vi "StringInputKeyboardSimulation_Tests.vi"(11 "error in":errorcluster) -> (15 "error out":errorcluster)   [LabVIEW 2016, in "DronaTest.lvlib"]
uses:
  DronaTest.lvlib
  APIs/Stimulus/KeyBoardSimulation/KeyboardSimulationForStringInput.vi
  APIs/Assert/AssertControlValue/Equal.vi
  <vilib>/addons/_JKI Toolkits/Caraya/classes/Test/Test.lvclass
  Drona.lvlib
  APIs/Assert/AssertControlValue/AssertControlValue.lvlib
  APIs/Stimulus/KeyBoardSimulation/KeyboardSimulation.lvlib
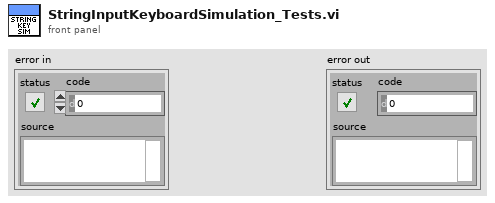
[diagram p1: front panel]
types:
  T1 = enum16{"Type all possible letters in keyboard", "TypeNegative25_ControlValueShouldBeNegative25", "Type255_ControlValueCoerceTo100", "TypeNegative257_ControlValueCoerceToNegative100"}[]
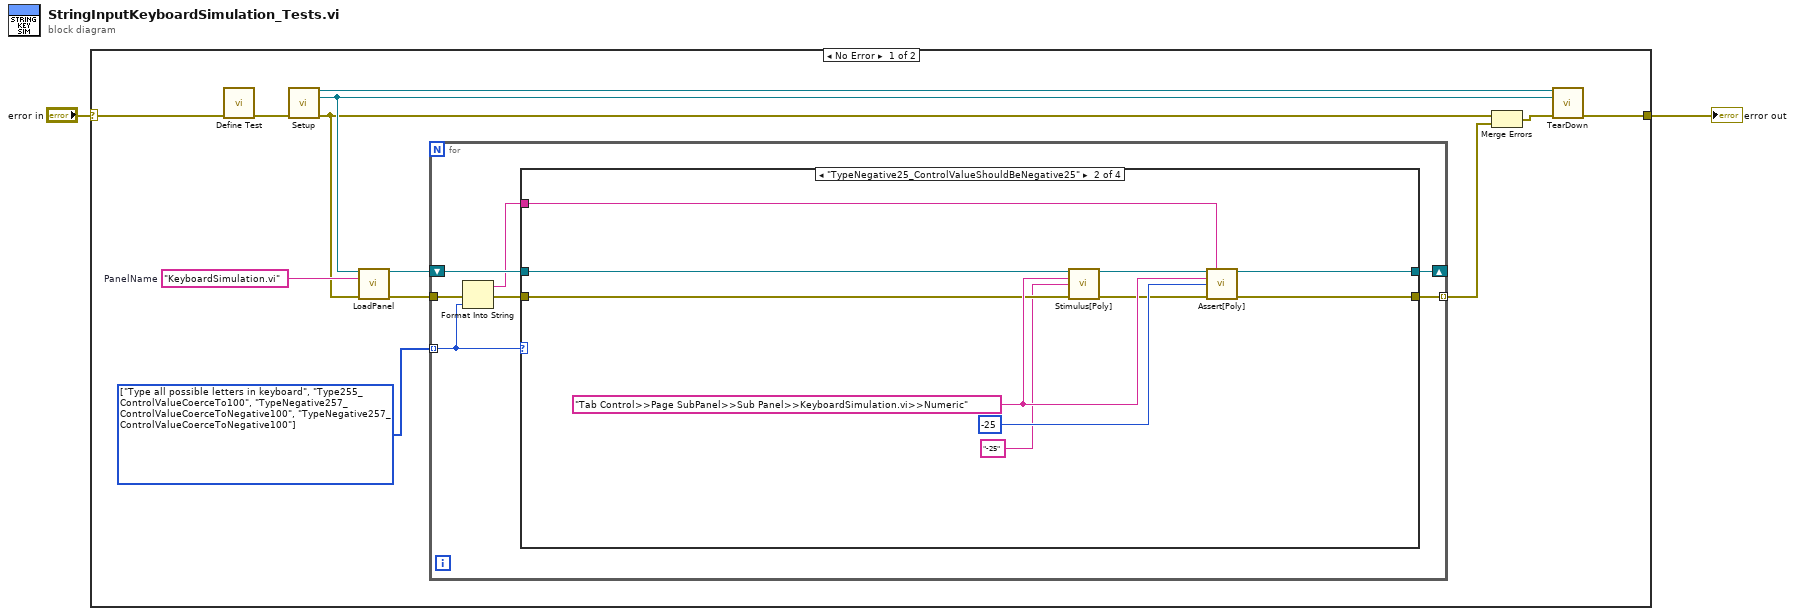
[diagram p0: block diagram]
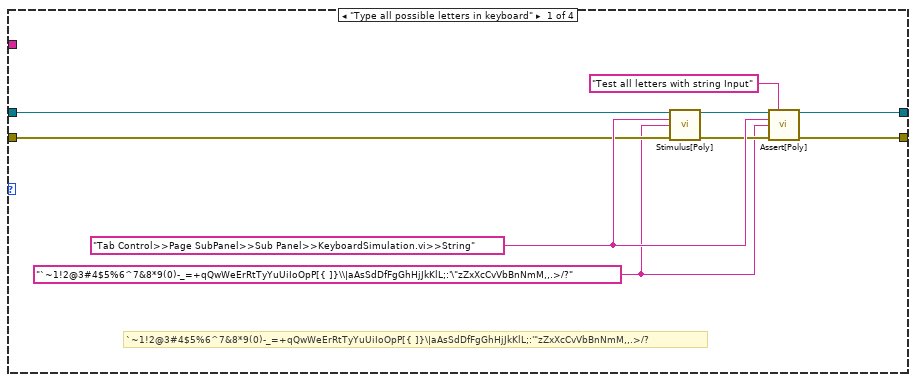
[diagram p2: hidden frame]
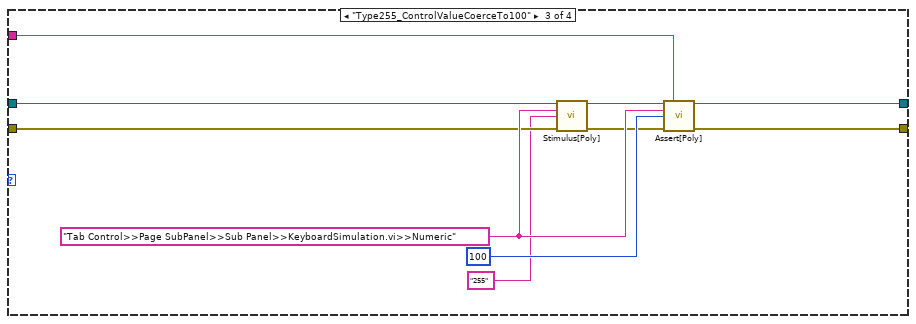
[diagram p3: hidden frame]
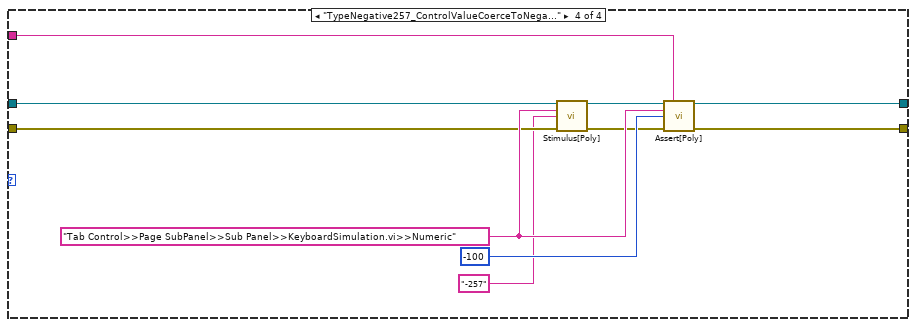
[diagram p4: hidden frame]
diagram:
  n1 = case shown="No Error" "error in" {
    selector: "error in" -> [w14 w61]
    tunnel: [w6 w61] -> w1
    frame No Error {
      w12 = T1 [enum."Type all possible letters in keyboard", enum."Type255_ControlValueCoerceTo100", enum."TypeNegative257_ControlValueCoerceToNegative100", enum."TypeNegative257_ControlValueCoerceToNegative100"] items=["Type all possible letters in keyboard", "TypeNegative25_ControlValueShouldBeNegative25", "Type255_ControlValueCoerceTo100", "TypeNegative257_ControlValueCoerceToNegative100"] ("TestCases")
      w13 = "KeyboardSimulation.vi"  # PanelName
      n2 = call <vilib>:"Define Test.vi"("error in (no error)"=w14) -> ("error out"=w8:errorcluster)  [unwired: 9 in, 1 out]
      n3 = call "Setup.vi"("error in"=w8) -> ("Application Ref"=w5:refnum<vi>, "VI out"=w4:refnum<vi>, "error out"=w3:errorcluster)  [unwired: 12 in]
      n4 = call "LoadPanel.vi"("VI in"=w4, "Item Name"=w13, "error in"=w3) -> ("VI out"=w9:refnum<vi>, "error out"=w11:errorcluster)  [unwired: 11 in]
      n5 = for {
        tunnel: w12 -> [w16] mode=indexing
        shift-right: [w20] -> _
        shift-left: w9 -> [w21]
        tunnel: w11 -> [w19]
        tunnel: [w18] -> w10 mode=indexing
        n6 = Format Into String(error in=w19, w16) -> (resulting string=w15:string, error out=w17:errorcluster)  [unwired: 2 in]
        n7 = case shown="\"TypeNegative25_ControlValueShouldBeNegative25\"" w16 {
          tunnel: [w27 w36 w46 w56] -> w18
          tunnel: w21 -> [w26 w34 w44 w54]
          tunnel: [w25 w35 w45 w55] -> w20
          tunnel: w17 -> [w24 w33 w43 w53]
          tunnel: w15 -> [_ w32 w42 w52]
          frame "Type all possible letters in keyboard" {
            w22 = "`~1!2@3#4$5%6^7&8*9(0)-_=+qQwWeErRtTyYuUiIoOpP[{ ]}\\|aAsSdDfFgGhHjJkKlL;:'\"zZxXcCvVbBnNmM,,.>/?" ("Control Path")
            w30 = "Tab Control>>Page SubPanel>>Sub Panel>>KeyboardSimulation.vi>>String" ("Control Path")
            # "`~1!2@3#4$5%6^7&8*9(0)-_=+qQwWeErRtTyYuUiIoOpP[{ ]}\\|aAsSdDfFgGhHjJkKlL;:'\"zZxXcCvVbBnNmM,,.>/?"
            n8 = call-poly "Stimulus[Poly].vi"("VI Reference In"=w26, "Control Path"=w30, "String Value"=w22, "Error In"=w24) -> ("VI Reference Out"=w29:refnum<vi>, "Error Out"=w28:errorcluster)  [unwired: 10 in]
            n9 = call-poly "Assert[Poly].vi"("VI Reference In"=w29, "Test Label"="Test all letters with string Input", "Control Path"=w30, "Control Value"=w22, "Error In"=w28) -> ("VI Reference Out"=w25:refnum<vi>, "Error Out"=w27:errorcluster)  [unwired: 8 in, 1 out]
          }
          frame "TypeNegative25_ControlValueShouldBeNegative25" {
            w39 = "Tab Control>>Page SubPanel>>Sub Panel>>KeyboardSimulation.vi>>Numeric" ("Control Path")
            n10 = call-poly "Stimulus[Poly].vi"("VI Reference In"=w34, "Control Path"=w39, "String Value"="-25" ("string"), "Error In"=w33) -> ("VI Reference Out"=w37:refnum<vi>, "Error Out"=w38:errorcluster)  [unwired: 10 in]
            n11 = call-poly "Assert[Poly].vi"("VI Reference In"=w37, "Test Label"=w32, "Control Path"=w39, "Control Value"=-25 ("Control Path"), "Error In"=w38) -> ("VI Reference Out"=w35:refnum<vi>, "Error Out"=w36:errorcluster)  [unwired: 8 in, 1 out]
          }
          frame "Type255_ControlValueCoerceTo100" {
            w49 = "Tab Control>>Page SubPanel>>Sub Panel>>KeyboardSimulation.vi>>Numeric" ("Control Path")
            n12 = call-poly "Stimulus[Poly].vi"("VI Reference In"=w44, "Control Path"=w49, "String Value"="255" ("string"), "Error In"=w43) -> ("VI Reference Out"=w47:refnum<vi>, "Error Out"=w48:errorcluster)  [unwired: 10 in]
            n13 = call-poly "Assert[Poly].vi"("VI Reference In"=w47, "Test Label"=w42, "Control Path"=w49, "Control Value"=100 ("Control Path"), "Error In"=w48) -> ("VI Reference Out"=w45:refnum<vi>, "Error Out"=w46:errorcluster)  [unwired: 8 in, 1 out]
          }
          frame "TypeNegative257_ControlValueCoerceToNegative100" {
            w59 = "Tab Control>>Page SubPanel>>Sub Panel>>KeyboardSimulation.vi>>Numeric" ("Control Path")
            n14 = call-poly "Stimulus[Poly].vi"("VI Reference In"=w54, "Control Path"=w59, "String Value"="-257" ("string"), "Error In"=w53) -> ("VI Reference Out"=w57:refnum<vi>, "Error Out"=w58:errorcluster)  [unwired: 10 in]
            n15 = call-poly "Assert[Poly].vi"("VI Reference In"=w57, "Test Label"=w52, "Control Path"=w59, "Control Value"=-100 ("Control Path"), "Error In"=w58) -> ("VI Reference Out"=w55:refnum<vi>, "Error Out"=w56:errorcluster)  [unwired: 8 in, 1 out]
          }
        }
      }
      n16 = Merge Errors(w3, w10) -> (w7:errorcluster)
      n17 = call "TearDown.vi"("Application Ref"=w5, "VI in"=w4, "error in (no error)"=w7) -> ("error out"=w6:errorcluster)  [unwired: 12 in]
    }
    frame Error {
    }
  }
  "error out" <- w1
